vi "Initialize Image.vi"(8 "error in":errorcluster, 11 "data type":T2) -> (0 "error out":errorcluster, 2 "Gray Image Out":T1, 3 "Color Image Out":T1)   [LabVIEW 2025, in "Automotive Vision.lvclass"]
doc: "Initialize the Imaq image reference."
uses:
  Automotive Vision.lvclass
  <instrlib>/FlexRIO/CSI-2/v2/Common/Types/LLP Data Type.ctl
  <vilib>/vision/Image Controls.llb/IMAQ Image.ctl
  Automotive Vision.lvclass/Automotive Vision.ctl
  <instrlib>/FlexRIO/CSI-2/v2/Common/NI CSI-2 API Common v2.lvlib
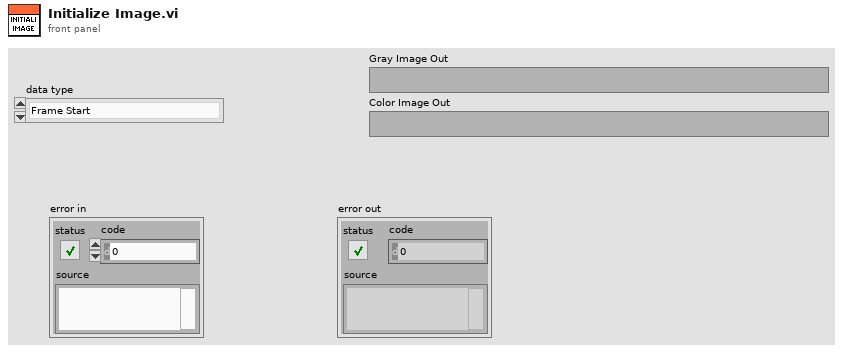
[diagram p1: front panel]
types:
  T1 = typedef "IMAQ Image.ctl" = refnum<image>
  T2 = typedef "NI CSI-2 API Common v2.lvlib/LLP Data Type.ctl" = enum8{"Frame Start", "Frame End", "Line Start", "Line End", "End of Transmission", "Reserved 0", "Reserved 1", "Reserved 2", "Generic Short Packet 1", "Generic Short Packet 2", "Generic Short Packet 3", "Generic Short Packet 4", "Generic Short Packet 5", "Generic Short Packet 6", "Generic Short Packet 7", "Generic Short Packet 8", "Null", "Blanking Data", "Embedded 8-bit non Image Data", "Generic Long Packet 1", "Generic Long Packet 2", "Generic Long Packet 3", "Generic Long Packet 4", "Reserved 3", "YUV420 8-bit", "YUV420 10-bit", "Legacy YUV420 8-bit", "Reserved 4", "YUV420 8-bit Chroma Shifted", "YUV420 10-bit Chroma Shifted", "YUV422 8-bit", "YUV422 10-bit", "RGB444", "RGB555", "RGB565", "RGB666", "RGB888", "Reserved 5", "Reserved 6", "RAW 24", "RAW 6", "RAW 7", "RAW 8", "RAW 10", "RAW 12", "RAW 14", "RAW 16", "RAW 20", "User Defined 8-bit Data 1", "User Defined 8-bit Data 2", "User Defined 8-bit Data 3", "User Defined 8-bit Data 4", "User Defined 8-bit Data 5", "User Defined 8-bit Data 6", "User Defined 8-bit Data 7", "User Defined 8-bit Data 8", "USL Command", "Reserved 7", "Reserved 8", "Reserved 9", "Reserved 10", "Reserved 11", "Reserved 12", "LRTE EPD Spacer"}
  T3 = typedef "Image Type" = u32
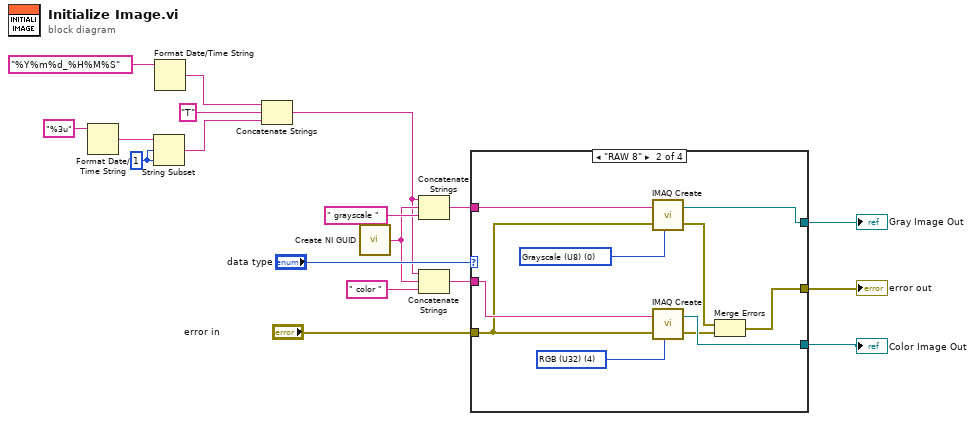
[diagram p0: block diagram]
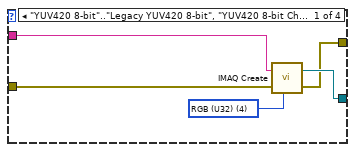
[diagram p2: hidden frame]
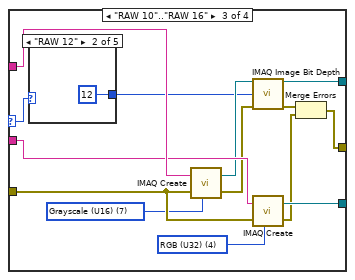
[diagram p3: hidden frame]
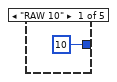
[diagram p4: hidden frame]
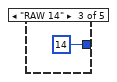
[diagram p5: hidden frame]
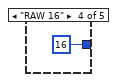
[diagram p6: hidden frame]
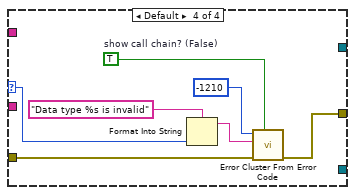
[diagram p8: hidden frame]
diagram:
  w1 = 1 ("offset (0)")
  n1 = Format Date/Time String(time format string (%c)="%3u") -> (date/time string=w5:string)  [unwired: 2 in]
  n2 = String Subset(string=w5, offset (0)=w1, length (rest)=w1) -> (substring=w2:string)
  n3 = Format Date/Time String(time format string (%c)="%Y%m%d_%H%M%S") -> (date/time string=w6:string)  [unwired: 2 in]
  n4 = Concatenate Strings(w6, "T" ("string"), w2) -> (w3:string)
  n5 = call <vilib>:"Create NI GUID.vi"() -> ("NI GUID"=w14:string)
  n6 = Concatenate Strings(w3, w14, " grayscale " ("Image Name")) -> (w17:string)
  n7 = Concatenate Strings(w3, w14, " color " ("Image Name")) -> (w16:string)
  n8 = case shown="\"RAW 8\"" "data type" {
    selector: "data type" -> [_ _ w41 w55]
    tunnel: w17 -> [_ w33 w47 _]
    tunnel: w16 -> [w22 w32 w46 _]
    tunnel: "error in" -> [w21 w31 w45 w53]
    tunnel: [w19 w30 w44 w52] -> w9
    tunnel: [w20 w29 w43 _] -> w10
    tunnel: [_ w28 w42 _] -> w11
    frame "YUV420 8-bit".."Legacy YUV420 8-bit", "YUV420 8-bit Chroma Shifted".."YUV422 10-bit", "RGB565".."RGB888" {
      w23 = T3 4 items=["Grayscale (U8)", "Grayscale (I16)", "Grayscale (SGL)", "Complex (CSG)", "RGB (U32)", "HSL (U32)", "RGB (U64)", "Grayscale (U16)"] ("Image Type")
      n9 = call "IMAQ Create"("Image Name"=w22, "Image Type"=w23, "error in (no error)"=w21) -> ("New Image"=w20:T1, "error out"=w19:errorcluster)  [unwired: 2 in]
    }
    frame "RAW 8" {
      w26 = T3 4 items=["Grayscale (U8)", "Grayscale (I16)", "Grayscale (SGL)", "Complex (CSG)", "RGB (U32)", "HSL (U32)", "RGB (U64)", "Grayscale (U16)"] ("Image Type")
      w27 = T3 0 items=["Grayscale (U8)", "Grayscale (I16)", "Grayscale (SGL)", "Complex (CSG)", "RGB (U32)", "HSL (U32)", "RGB (U64)", "Grayscale (U16)"] ("Image Type")
      n10 = call "IMAQ Create"("Image Name"=w33, "Image Type"=w27, "error in (no error)"=w31) -> ("New Image"=w28:T1, "error out"=w24:errorcluster)  [unwired: 2 in]
      n11 = call "IMAQ Create"("Image Name"=w32, "Image Type"=w26, "error in (no error)"=w31) -> ("New Image"=w29:T1, "error out"=w25:errorcluster)  [unwired: 2 in]
      n12 = Merge Errors(w24, w25) -> (w30:errorcluster)
    }
    frame "RAW 10".."RAW 16" {
      w39 = T3 4 items=["Grayscale (U8)", "Grayscale (I16)", "Grayscale (SGL)", "Complex (CSG)", "RGB (U32)", "HSL (U32)", "RGB (U64)", "Grayscale (U16)"] ("Image Type")
      w40 = T3 7 items=["Grayscale (U8)", "Grayscale (I16)", "Grayscale (SGL)", "Complex (CSG)", "RGB (U32)", "HSL (U32)", "RGB (U64)", "Grayscale (U16)"] ("Image Type")
      n13 = case shown="\"RAW 12\"" w41 {
        tunnel: [u32 10 ("Bit Depth (0)") u32 12 ("Bit Depth (0)") u32 14 ("Bit Depth (0)") u32 16 ("Bit Depth (0)") _] -> w34
        frame "RAW 10" {
        }
        frame "RAW 12" {
        }
        frame "RAW 14" {
        }
        frame "RAW 16" {
        }
        frame Default {
        }
      }
      n14 = call "IMAQ Create"("Image Name"=w47, "Image Type"=w40, "error in (no error)"=w45) -> ("New Image"=w37:T1, "error out"=w36:errorcluster)  [unwired: 2 in]
      n15 = call "IMAQ Image Bit Depth"("Image"=w37, "Bit Depth (0)"=w34, "error in (no error)"=w36) -> ("Image Out"=w42:T1, "error out"=w35:errorcluster)  [unwired: 10 in, 1 out]
      n16 = call "IMAQ Create"("Image Name"=w46, "Image Type"=w39, "error in (no error)"=w45) -> ("New Image"=w43:T1, "error out"=w38:errorcluster)  [unwired: 2 in]
      n17 = Merge Errors(w35, w38) -> (w44:errorcluster)
    }
    frame Default {
      w57 = TRUE  # show call chain? (False)
      n18 = Format Into String(format string="Data type %s is invalid" ("error message (\"\")"), w55) -> (resulting string=w54:string)  [unwired: 2 in, 1 out]
      n19 = call <vilib>:"Error Cluster From Error Code.vi"("show call chain? (False)"=w57, "error in (no error)"=w53, "error message (\"\")"=w54, "error code (0)"=-1210) -> ("error out"=w52:errorcluster)  [unwired: 5 in]
    }
  }
  "Gray Image Out" <- w11
  "Color Image Out" <- w10
  "error out" <- w9
